vi "Measurement Logic.vi"() -> ()   [LabVIEW 2021, in "Load Transient_Channel Ganging.lvlib"]
uses:
  Load Transient_Channel Ganging.lvlib
  <vilib>/Plug-In SDKs/Measurements/Measure Call Context/Measure Call Context.lvclass
  Measurement Configuration.ctl
  Measurement Results.ctl
  <instrlib>/niDCPower/nidcpower.llb/niDCPower Source Mode.ctl
  <instrlib>/niDCPower/nidcpower.llb/niDCPower Output Function.ctl
  <instrlib>/niDCPower/nidcpower.llb/niDCPower Wait For Event - Event.ctl
  shared subVIs/ctl/NIDCPower_channel_ganging - ctl - channel mode.ctl
panel:
  out "measurement results":T1
  in  "measurement configuration":T2={"Source system configuration"=enum."Parallel", "Source voltage level range"=1.2, "Source limit symmetry"=enum."Asymmetric", "Source current limit range"=32.0, "Source current limit low"=64.0, "Source current limit high"=64.0, "Load system configuration"=enum."Series", "Source transient response"=-32, "Source sense"=-64, "Source voltage level"=-64.0, "Source master resource name"="Lorem ipsum dolor sit", "Load master resource name"="Lorem ipsum dolor sit", "Source slave resource names"=["", ""], "Load slave resource names"=["", ""], "Source voltage gain bandwidth"=1.0, "Source voltage compensation frequency"=1.0, "Source voltage pole-zero ratio"=2.0, "Load sample rate"=1800000.0, "Load current level range"=80.0, "Load sense"=1009, "Load current set point 1"=4.0, "Load current set point 2"=14.0, "Load current rising slew rate"=24.0, "Load current falling slew rate"=24.0, "Load limit symmetry"=enum."Symmetric", "Load voltage limit range"=6.0, "Load voltage limit low"=0.0, "Load voltage limit high"=inf, "Load transient response"=1038, "Load current gain bandwidth"=14000.0, "Load current compensation frequency"=180000.0, "Load current pole-zero ratio"=0.3, "DUT setup time"=1.0, "Nominal output voltage"=1.0, "Level dwell time"=0.005} {"Load transient response" items=["Slow"=1041, "Normal"=1038, "Fast"=1039, "Custom"=1042]; "Load current rising slew rate" format="%#_6p"; "Load current set point 2" format="%#_6p"; "Load current set point 1" format="%#_6p"; "Load sense" items=["Symmetric", "Asymmetric"]; "Load current level range" format="%#_6p"; "Source sense" items=["Local"=1008, "Remote"=1009]; "Source transient response" items=["Slow"=1041, "Normal"=1038, "Fast"=1039, "Custom"=1042]; "Source current limit low" format="%#_6p"}
  out "measure call context out":refnum<class "Measure Call Context.lvclass">
  in  "measure call context in":refnum<class "Measure Call Context.lvclass">
  out "error out":errorcluster
  in  "error in":errorcluster
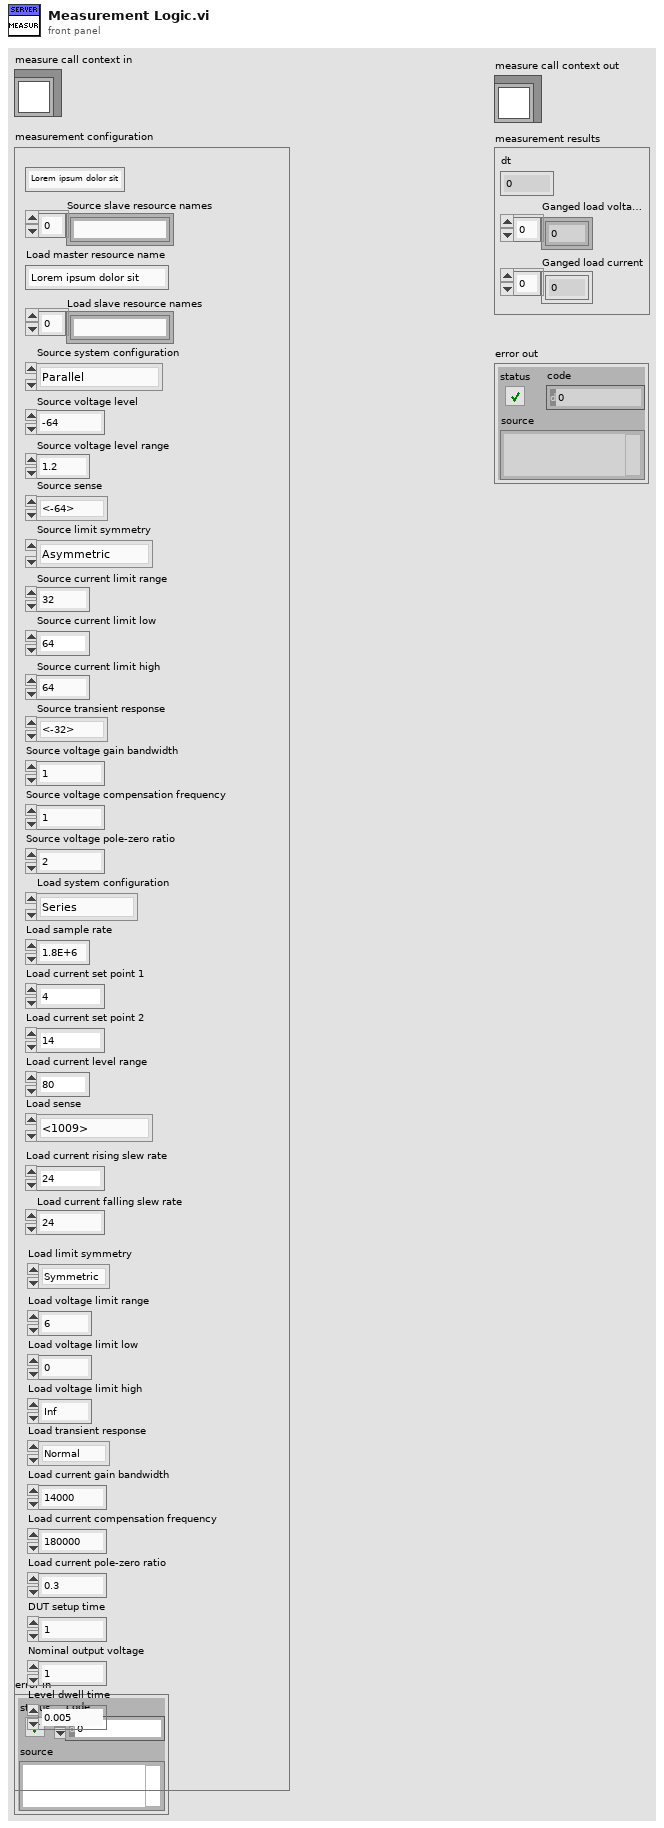
[diagram p1: front panel]
types:
  T1 = typedef "Load Transient_Channel Ganging.lvlib/Measurement Results.ctl" = cluster{"dt":dbl, "Ganged load voltages":dbl[], "Ganged load current":dbl[]}
  T2 = typedef "Load Transient_Channel Ganging.lvlib/Measurement Configuration.ctl" = cluster{"Source system configuration":enum32{"Series", "Parallel", "Manual"}, "Source voltage level range":dbl, "Source limit symmetry":enum32{"Symmetric", "Asymmetric"}, "Source current limit range":dbl, "Source current limit low":dbl, "Source current limit high":dbl, "Load system configuration":enum32{"Series", "Parallel", "Manual"}, "Source transient response":i32, "Source sense":i32, "Source voltage level":dbl, "Source master resource name":string, "Load master resource name":string, "Source slave resource names":string[], "Load slave resource names":string[], "Source voltage gain bandwidth":dbl, "Source voltage compensation frequency":dbl, "Source voltage pole-zero ratio":dbl, "Load sample rate":dbl, "Load current level range":dbl, "Load sense":i32, "Load current set point 1":dbl, "Load current set point 2":dbl, "Load current rising slew rate":dbl, "Load current falling slew rate":dbl, "Load limit symmetry":enum32{"Symmetric", "Asymmetric"}, "Load voltage limit range":dbl, "Load voltage limit low":dbl, "Load voltage limit high":dbl, "Load transient response":i32, "Load current gain bandwidth":dbl, "Load current compensation frequency":dbl, "Load current pole-zero ratio":dbl, "DUT setup time":dbl, "Nominal output voltage":dbl, "Level dwell time":dbl}
  T3 = typedef "NIDCPower_channel_ganging - ctl - channel mode.ctl" = enum32{"Master", "Slave", "Slave - Inverted"}
  T4 = typedef "niDCPower Wait For Event - Event.ctl" = i32
  T5 = typedef "niDCPower Output Function.ctl" = i32
  T6 = typedef "niDCPower Source Mode.ctl" = i32
  T7 = typedef "NIDCPower_channel_ganging - ctl - channel def.ctl" = cluster{"resource name":refnum<k15>, "channels":string, "Channel Mode":T3}
  T8 = typedef "NIDCPower_channel_ganging - ctl - ganged session.ctl" = cluster{"Ganged Config":T9, "Session List":refnum<k15>[], "Session Mode":T3[], "Channel":string[]}
  T9 = typedef "NIDCPower_channel_ganging - ctl - ganged config.ctl" = enum32{"Series", "Parallel", "Manual"}
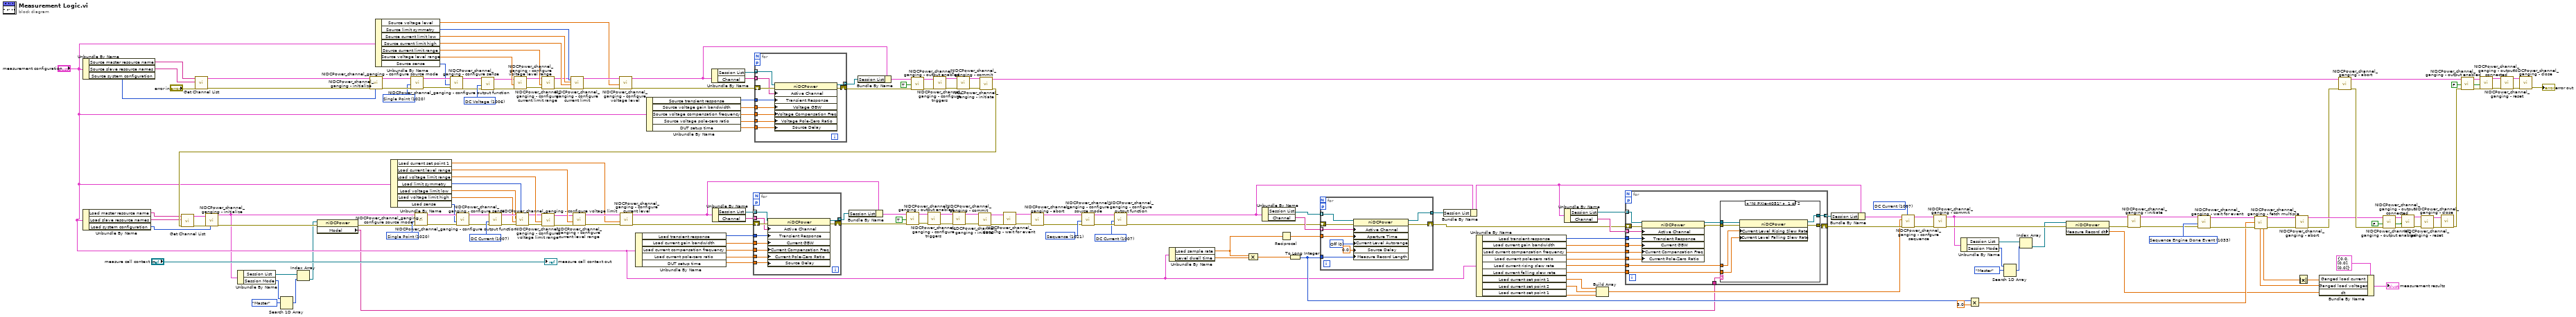
[diagram p0: block diagram]
diagram:
  w42 = FALSE ("output enabled")
  w41 = FALSE ("output enabled")
  w56 = T4 1033 items=["Source Complete Event"=1030, "Measure Complete Event"=1031, "Sequence Iteration Complete Event"=1032, "Sequence Engine Done Event"=1033, "Pulse Complete Event"=1051, "Ready For Pulse Trigger Event"=1052] ("event")
  w72 = T5 1007 items=["DC Voltage"=1006, "DC Current"=1007, "Pulse Voltage"=1049, "Pulse Current"=1050] ("output function")
  w95 = T6 1021 items=["Single Point"=1020, "Sequence"=1021] ("source mode")
  w94 = T5 1007 items=["DC Voltage"=1006, "DC Current"=1007, "Pulse Voltage"=1049, "Pulse Current"=1050] ("output function")
  w155 = T5 1007 items=["DC Voltage"=1006, "DC Current"=1007, "Pulse Voltage"=1049, "Pulse Current"=1050] ("output function")
  w168 = T5 1006 items=["DC Voltage"=1006, "DC Current"=1007, "Pulse Voltage"=1049, "Pulse Current"=1050] ("output function")
  w185 = T6 1020 items=["Single Point"=1020, "Sequence"=1021] ("source mode")
  w186 = T6 1020 items=["Single Point"=1020, "Sequence"=1021] ("source mode")
  n1 = Unbundle By Name("measurement configuration") -> ("Source master resource name"=w114:string, "Source slave resource names"=w113:string[], "Source system configuration"=w170:enum32{"Series", "Parallel", "Manual"})
  n2 = Unbundle By Name("measurement configuration") -> ("Load master resource name"=w110:string, "Load slave resource names"=w109:string[], "Load system configuration"=w169:enum32{"Series", "Parallel", "Manual"})
  n3 = call "Get Channel List.vi"("error in (no error)"="error in", "Slave resource names"=w113, "Master resouce name"=w114) -> ("error out"=w115:errorcluster, "Channel List"=w116:T7[])  [unwired: 7 in]
  n4 = call "NIDCPower_channel_ganging - initialize.vi"("Ganged Config"=w170, "error in (no error)"=w115, "Channel List"=w116) -> ("error out"=w187:errorcluster, "Ganged Session Out"=w188:T8)  [unwired: 7 in]
  n5 = Unbundle By Name("measurement configuration") -> ("Source voltage level"=w98:dbl, "Source limit symmetry"=w176:enum32{"Symmetric", "Asymmetric"}, "Source current limit low"=w177:dbl, "Source current limit high"=w178:dbl, "Source current limit range"=w179:dbl, "Source voltage level range"=w180:dbl, "Source sense"=w117:i32)
  n6 = Unbundle By Name("measurement configuration") -> ("Load current set point 1"=w119:dbl, "Load current level range"=w171:dbl, "Load voltage limit range"=w172:dbl, "Load limit symmetry"=w175:enum32{"Symmetric", "Asymmetric"}, "Load voltage limit low"=w174:dbl, "Load voltage limit high"=w173:dbl, "Load sense"=w118:i32)
  n7 = call "NIDCPower_channel_ganging - configure source mode.vi"("error in (no error)"=w187, "source mode"=w186, "Ganged Session In"=w188) -> ("error out"=w153:errorcluster, "Ganged Session Out"=w154:T8)  [unwired: 7 in]
  n8 = call "NIDCPower_channel_ganging - configure sense.vi"("error in (no error)"=w153, "sense"=w117, "Ganged Session In"=w154) -> ("error out"=w151:errorcluster, "Ganged Session Out"=w152:T8)  [unwired: 7 in]
  n9 = call "NIDCPower_channel_ganging - configure output function.vi"("error in (no error)"=w151, "output function"=w168, "Ganged Session In"=w152) -> ("error out"=w149:errorcluster, "Ganged Session Out"=w150:T8)  [unwired: 7 in]
  n10 = call "NIDCPower_channel_ganging - configure voltage level range.vi"("error in (no error)"=w149, "voltage level range"=w180, "Ganged Session In"=w150) -> ("error out"=w164:errorcluster, "Ganged Session Out"=w167:T8)  [unwired: 7 in]
  n11 = call "NIDCPower_channel_ganging - configure current limit range.vi"("error in (no error)"=w164, "current limit range"=w179, "Ganged Session In"=w167) -> ("error out"=w163:errorcluster, "Ganged Session Out"=w166:T8)  [unwired: 7 in]
  n12 = call "NIDCPower_channel_ganging - configure current limit.vi"("Limit Symmetry"=w176, "error in (no error)"=w163, "Current limit/hi"=w178, "Current limit lo"=w177, "Ganged Session In"=w166) -> ("error out"=w162:errorcluster, "Ganged Session Out"=w165:T8)  [unwired: 5 in]
  n13 = call "NIDCPower_channel_ganging - configure voltage level.vi"("error in (no error)"=w162, "voltage level"=w98, "Ganged Session In"=w165) -> ("error out"=w127:errorcluster, "Ganged Session Out"=w61:T8)  [unwired: 7 in]
  n14 = Unbundle By Name("measurement configuration") -> ("Load transient response"=w107:i32, "Load current gain bandwidth"=w101:dbl, "Load current compensation frequency"=w100:dbl, "Load current pole-zero ratio"=w99:dbl, "DUT setup time"=w106:dbl)
  n15 = Unbundle By Name("measurement configuration") -> ("Source transient response"=w108:i32, "Source voltage gain bandwidth"=w104:dbl, "Source voltage compensation frequency"=w103:dbl, "Source voltage pole-zero ratio"=w102:dbl, "DUT setup time"=w105:dbl)
  n16 = Unbundle By Name(w61) -> ("Session List"=w125:refnum<k15>[], "Channel"=w124:string[])
  n17 = for {
    tunnel: [w199] -> w60 mode=indexing
    shift-right: [w197] -> w126
    shift-left: w127 -> [w198]
    workers-P: _ -> [_]
    tunnel: w125 -> [w196] mode=indexing
    tunnel: w124 -> [w195] mode=indexing
    tunnel: w108 -> [w194]
    tunnel: w105 -> [w193]
    tunnel: w104 -> [w192]
    tunnel: w103 -> [w191]
    tunnel: w102 -> [w190]
    n18 = property class="niDCPower"(reference=w196, error in=w198, "Active Channel"=w195, "Transient Response"=w194, "Voltage GBW"=w192, "Voltage Compensation Freq"=w191, "Voltage Pole-Zero Ratio"=w190, "Source Delay"=w193) -> (reference out=w199:refnum<k15>, error out=w197:errorcluster)
  }
  n19 = Bundle By Name(cluster=w61, "Session List"=w60) -> (w59:T8)
  n20 = call "NIDCPower_channel_ganging - output enabled.vi"("error in (no error)"=w126, "output enabled"=TRUE, "Ganged Session In"=w59) -> ("error out"=w130:errorcluster, "Ganged Session Out"=w131:T8)  [unwired: 7 in]
  n21 = call "NIDCPower_channel_ganging - configure triggers.vi"("error in (no error)"=w130, "Ganged Session In"=w131) -> ("error out"=w128:errorcluster, "Ganged Session Out"=w129:T8)  [unwired: 8 in]
  n22 = call "NIDCPower_channel_ganging - commit.vi"("error in (no error)"=w128, "Ganged Session In"=w129) -> ("error out"=w137:errorcluster, "Ganged Session Out"=w136:T8)  [unwired: 8 in]
  n23 = call "NIDCPower_channel_ganging - initiate.vi"("error in (no error)"=w137, "Ganged Session In"=w136) -> ("error out"=w138:errorcluster, "Ganged Session Out"=w30:T8)  [unwired: 8 in]
  n24 = call "Get Channel List.vi"("error in (no error)"=w138, "Slave resource names"=w109, "Master resouce name"=w110) -> ("error out"=w112:errorcluster, "Channel List"=w111:T7[])  [unwired: 7 in]
  n25 = call "NIDCPower_channel_ganging - initialize.vi"("Ganged Config"=w169, "error in (no error)"=w112, "Channel List"=w111) -> ("error out"=w6:errorcluster, "Ganged Session Out"=w3:T8)  [unwired: 7 in]
  n26 = Unbundle By Name(w3) -> ("Session List"=w10:refnum<k15>[], "Session Mode"=w9:T3[])
  n27 = Search 1D Array(1D array=w9, element=NIDCPower_channel_ganging_-_ctl_-_channel_mode."Master") -> (index of element=w7:i32)  [unwired: 1 in]
  n28 = Index Array(array=w10, index=w7) -> (element=w5:refnum<k15>)
  n29 = property class="niDCPower"(reference=w5, error in=w6) -> (error out=w4:errorcluster, "Model"=w2:string)  [unwired: 1 out]
  n30 = call "NIDCPower_channel_ganging - configure source mode.vi"("error in (no error)"=w4, "source mode"=w185, "Ganged Session In"=w3) -> ("error out"=w147:errorcluster, "Ganged Session Out"=w148:T8)  [unwired: 7 in]
  n31 = call "NIDCPower_channel_ganging - configure sense.vi"("error in (no error)"=w147, "sense"=w118, "Ganged Session In"=w148) -> ("error out"=w145:errorcluster, "Ganged Session Out"=w146:T8)  [unwired: 7 in]
  n32 = call "NIDCPower_channel_ganging - configure output function.vi"("error in (no error)"=w145, "output function"=w155, "Ganged Session In"=w146) -> ("error out"=w183:errorcluster, "Ganged Session Out"=w184:T8)  [unwired: 7 in]
  n33 = call "NIDCPower_channel_ganging - configure voltage limit.vi"("Limit Symmetry"=w175, "error in (no error)"=w183, "voltage limit/hi"=w173, "voltage limit lo"=w174, "Ganged Session In"=w184) -> ("error out"=w160:errorcluster, "Ganged Session Out"=w161:T8)  [unwired: 5 in]
  n34 = call "NIDCPower_channel_ganging - configure voltage limit range.vi"("error in (no error)"=w160, "voltage level range"=w172, "Ganged Session In"=w161) -> ("error out"=w158:errorcluster, "Ganged Session Out"=w159:T8)  [unwired: 7 in]
  n35 = call "NIDCPower_channel_ganging - configure current level range.vi"("error in (no error)"=w158, "current level range"=w171, "Ganged Session In"=w159) -> ("error out"=w156:errorcluster, "Ganged Session Out"=w157:T8)  [unwired: 7 in]
  n36 = call "NIDCPower_channel_ganging - configure current level.vi"("error in (no error)"=w156, "current level"=w119, "Ganged Session In"=w157) -> ("error out"=w123:errorcluster, "Ganged Session Out"=w64:T8)  [unwired: 7 in]
  n37 = Unbundle By Name(w64) -> ("Session List"=w121:refnum<k15>[], "Channel"=w120:string[])
  n38 = for {
    tunnel: [w209] -> w62 mode=indexing
    shift-right: [w207] -> w122
    shift-left: w123 -> [w208]
    workers-P: _ -> [_]
    tunnel: w121 -> [w206] mode=indexing
    tunnel: w120 -> [w205] mode=indexing
    tunnel: w107 -> [w204]
    tunnel: w106 -> [w203]
    tunnel: w101 -> [w202]
    tunnel: w100 -> [w201]
    tunnel: w99 -> [w200]
    n39 = property class="niDCPower"(reference=w206, error in=w208, "Active Channel"=w205, "Transient Response"=w204, "Current GBW"=w202, "Current Compensation Freq"=w201, "Current Pole-Zero Ratio"=w200, "Source Delay"=w203) -> (reference out=w209:refnum<k15>, error out=w207:errorcluster)
  }
  n40 = Bundle By Name(cluster=w64, "Session List"=w62) -> (w63:T8)
  n41 = call "NIDCPower_channel_ganging - output enabled.vi"("error in (no error)"=w122, "output enabled"=TRUE, "Ganged Session In"=w63) -> ("error out"=w134:errorcluster, "Ganged Session Out"=w135:T8)  [unwired: 7 in]
  n42 = call "NIDCPower_channel_ganging - configure triggers.vi"("error in (no error)"=w134, "Ganged Session In"=w135) -> ("error out"=w132:errorcluster, "Ganged Session Out"=w133:T8)  [unwired: 8 in]
  n43 = call "NIDCPower_channel_ganging - commit.vi"("error in (no error)"=w132, "Ganged Session In"=w133) -> ("error out"=w143:errorcluster, "Ganged Session Out"=w144:T8)  [unwired: 8 in]
  n44 = call "NIDCPower_channel_ganging - initiate.vi"("error in (no error)"=w143, "Ganged Session In"=w144) -> ("error out"=w141:errorcluster, "Ganged Session Out"=w142:T8)  [unwired: 8 in]
  n45 = call "NIDCPower_channel_ganging - wait for event.vi"("error in (no error)"=w141, "Ganged Session in"=w142) -> ("error out"=w139:errorcluster, "Ganged Session Out"=w140:T8)  [unwired: 8 in]
  n46 = call "NIDCPower_channel_ganging - abort.vi"("error in (no error)"=w139, "Ganged Session In"=w140) -> ("error out"=w93:errorcluster, "Ganged Session Out"=w92:T8)  [unwired: 8 in]
  n47 = call "NIDCPower_channel_ganging - configure source mode.vi"("error in (no error)"=w93, "source mode"=w95, "Ganged Session In"=w92) -> ("error out"=w97:errorcluster, "Ganged Session Out"=w96:T8)  [unwired: 7 in]
  n48 = call "NIDCPower_channel_ganging - configure output function.vi"("error in (no error)"=w97, "output function"=w94, "Ganged Session In"=w96) -> ("error out"=w89:errorcluster, "Ganged Session Out"=w66:T8)  [unwired: 7 in]
  n49 = Unbundle By Name("measurement configuration") -> ("Load sample rate"=w86:dbl, "Level dwell time"=w85:dbl)
  n50 = Compound Arithmetic op=MULTIPLY(w86, w85) -> (w87:dbl)
  n51 = Unbundle By Name(w66) -> ("Session List"=w91:refnum<k15>[], "Channel"=w90:string[])
  n52 = Reciprocal(x=w86) -> (1/x=w88:dbl)
  n53 = To Long Integer(number=w87) -> (32bit integer=w27:i32)
  n54 = for {
    tunnel: [w218] -> w67 mode=indexing
    shift-right: [w216] -> w78
    shift-left: w89 -> [w217]
    workers-P: _ -> [_]
    tunnel: w91 -> [w215] mode=indexing
    tunnel: w90 -> [w214] mode=indexing
    tunnel: w88 -> [w213]
    tunnel: w27 -> [w211]
    w210 = 0 items=["Off", "On"] ("Source:DC Current:Current Level Autorange")
    n55 = property class="niDCPower"(reference=w215, error in=w217, "Active Channel"=w214, "Aperture Time"=w213, "Current Level Autorange"=w210, "Source Delay"=0.0 ("Source:Advanced:Source Delay"), "Measure Record Length"=w211) -> (reference out=w218:refnum<k15>, error out=w216:errorcluster)
  }
  n56 = Bundle By Name(cluster=w66, "Session List"=w67) -> (w65:T8)
  n57 = Unbundle By Name("measurement configuration") -> ("Load transient response"=w82:i32, "Load current gain bandwidth"=w81:dbl, "Load current compensation frequency"=w80:dbl, "Load current pole-zero ratio"=w79:dbl, "Load current rising slew rate"=w12:dbl, "Load current falling slew rate"=w11:dbl, "Load current set point 1"=w76:dbl, "Load current set point 2"=w75:dbl, "Load current set point 1"=w74:dbl)
  n58 = Unbundle By Name(w65) -> ("Session List"=w84:refnum<k15>[], "Channel"=w83:string[])
  n59 = Build Array(w76, w75, w74) -> (w73:dbl[])
  n60 = for {
    tunnel: [w222] -> w69 mode=indexing
    shift-right: [w223] -> w77
    shift-left: w78 -> [w232]
    workers-P: _ -> [_]
    tunnel: w84 -> [w231] mode=indexing
    tunnel: w83 -> [w230] mode=indexing
    tunnel: w82 -> [w229]
    tunnel: w81 -> [w228]
    tunnel: w80 -> [w227]
    tunnel: w79 -> [w226]
    tunnel: w12 -> [w220]
    tunnel: w11 -> [w219]
    tunnel: w2 -> [w221]
    n61 = property class="niDCPower"(reference=w231, error in=w232, "Active Channel"=w230, "Transient Response"=w229, "Current GBW"=w228, "Current Compensation Freq"=w227, "Current Pole-Zero Ratio"=w226) -> (reference out=w224:refnum<k15>, error out=w225:errorcluster)
    n62 = case shown="\"NI PXIe-4051\"" w221 {
      tunnel: w225 -> [w238 w240]
      tunnel: w224 -> [w237 w239]
      tunnel: [w233 w240] -> w223
      tunnel: [w234 w239] -> w222
      tunnel: w220 -> [w236 _]
      tunnel: w219 -> [w235 _]
      frame "NI PXIe-4051" {
        n63 = property class="niDCPower"(reference=w237, error in=w238, "Current Level Rising Slew Rate"=w236, "Current Level Falling Slew Rate"=w235) -> (reference out=w234:refnum<k15>, error out=w233:errorcluster)
      }
      frame "NI PXIe-4139", Default {
      }
    }
  }
  n64 = Bundle By Name(cluster=w65, "Session List"=w69) -> (w68:T8)
  n65 = call "NIDCPower_channel_ganging - confgure sequence.vi"("output function"=w72, "error in (no error)"=w77, "Values"=w73, "Ganged Session In"=w68) -> ("error out"=w71:errorcluster, "Ganged Session Out"=w70:T8)  [unwired: 6 in]
  n66 = call "NIDCPower_channel_ganging - commit.vi"("error in (no error)"=w71, "Ganged Session In"=w70) -> ("error out"=w58:errorcluster, "Ganged Session Out"=w57:T8)  [unwired: 8 in]
  n67 = Unbundle By Name(w57) -> ("Session List"=w25:refnum<k15>[], "Session Mode"=w24:T3[])
  n68 = Multiply(x=w27, y=3.0) -> (x*y=w29:dbl)
  n69 = Search 1D Array(1D array=w24, element=NIDCPower_channel_ganging_-_ctl_-_channel_mode."Master") -> (index of element=w22:i32)  [unwired: 1 in]
  n70 = Index Array(array=w25, index=w22) -> (element=w26:refnum<k15>)
  n71 = property class="niDCPower"(reference=w26, error in=w58) -> (error out=w54:errorcluster, "Measure Record dt"=w13:dbl)  [unwired: 1 out]
  n72 = call "NIDCPower_channel_ganging - initiate.vi"("error in (no error)"=w54, "Ganged Session In"=w57) -> ("error out"=w53:errorcluster, "Ganged Session Out"=w55:T8)  [unwired: 8 in]
  n73 = call "NIDCPower_channel_ganging - wait for event.vi"("error in (no error)"=w53, "event"=w56, "Ganged Session in"=w55) -> ("error out"=w51:errorcluster, "Ganged Session Out"=w52:T8)  [unwired: 7 in]
  n74 = call "NIDCPower_channel_ganging - fetch multiple.vi"("Ganged Session In"=w52, "Count"=w29, "error in (no error)"=w51) -> ("Ganged Voltage Measurement"=w15:dbl[], "Ganged Current Measurement"=w14:dbl[], "Ganged Session Out"=w32:T8, "error out"=w31:errorcluster)  [unwired: 5 in, 4 out]
  n75 = call "NIDCPower_channel_ganging - abort.vi"("error in (no error)"=w31, "Ganged Session In"=w32) -> ("error out"=w16:errorcluster, "Ganged Session Out"=w47:T8)  [unwired: 8 in]
  n76 = Absolute Value(x=w14) -> (abs(x)=w1:dbl[])
  n77 = Bundle By Name(cluster=T1 {"dt"=0.0, "Ganged load voltages"=[0.0], "Ganged load current"=[0.0]} ("measurement results"), "Ganged load current"=w1, "Ganged load voltages"=w15, "dt"=w13) -> (→"measurement results":T1)
  n78 = call "NIDCPower_channel_ganging - abort.vi"("error in (no error)"=w16, "Ganged Session In"=w30) -> ("error out"=w50:errorcluster, "Ganged Session Out"=w43:T8)  [unwired: 8 in]
  n79 = call "NIDCPower_channel_ganging - output enabled.vi"("error in (no error)"=w50, "output enabled"=w42, "Ganged Session In"=w47) -> ("error out"=w48:errorcluster, "Ganged Session Out"=w49:T8)  [unwired: 7 in]
  n80 = call "NIDCPower_channel_ganging - output connected.vi"("error in (no error)"=w48, "output enabled"=w42, "Ganged Session In"=w49) -> ("error out"=w40:errorcluster, "Ganged Session Out"=w39:T8)  [unwired: 7 in]
  n81 = call "NIDCPower_channel_ganging - reset.vi"("error in (no error)"=w40, "Ganged Session In"=w39) -> ("error out"=w37:errorcluster, "Ganged Session Out"=w38:T8)  [unwired: 8 in]
  n82 = call "NIDCPower_channel_ganging - close.vi"("error in (no error)"=w37, "Ganged Session In"=w38) -> ("error out"=w44:errorcluster)  [unwired: 9 in]
  n83 = call "NIDCPower_channel_ganging - output enabled.vi"("error in (no error)"=w44, "output enabled"=w41, "Ganged Session In"=w43) -> ("error out"=w46:errorcluster, "Ganged Session Out"=w45:T8)  [unwired: 7 in]
  n84 = call "NIDCPower_channel_ganging - output connected.vi"("error in (no error)"=w46, "output enabled"=w41, "Ganged Session In"=w45) -> ("error out"=w35:errorcluster, "Ganged Session Out"=w36:T8)  [unwired: 7 in]
  n85 = call "NIDCPower_channel_ganging - reset.vi"("error in (no error)"=w35, "Ganged Session In"=w36) -> ("error out"=w33:errorcluster, "Ganged Session Out"=w34:T8)  [unwired: 8 in]
  n86 = call "NIDCPower_channel_ganging - close.vi"("error in (no error)"=w33, "Ganged Session In"=w34) -> ("error out"=→"error out":errorcluster)  [unwired: 9 in]
  "measure call context out" <- "measure call context in"
